vi "Create Channel.vi"(3 "no of points":u8, 5 "WheelID (if need)":u8, 7 "PlayerID":u8=1, 8 "error in (no error)":errorcluster, 9 "Channel":T2, 10 "RDB Signalname":string, 11 "Item Ref in":T1 format="%.0x") -> (0 "error out":errorcluster)   [LabVIEW 2023, in "Vires VTD System Explorer.lvlib"]
uses:
  Vires VTD System Explorer.lvlib
  <vilib>/NI VeriStand/Custom Device API/Custom Device Channel.ctl
  <vilib>/NI VeriStand/Custom Device API/Custom Device Channel Type.ctl
  <vilib>/NI VeriStand/Custom Device API/Custom Device Item Ref.ctl
  <vilib>/xnet/xnet.llb/XNET String To IO Name (Signal).vi
  Shared/Constants.vi
  <vilib>/NI VeriStand/Custom Device API/Custom Device API.lvlib
  Shared/Vires VTD Shared.lvlib
  <resource>/objmgr/xnet.rc
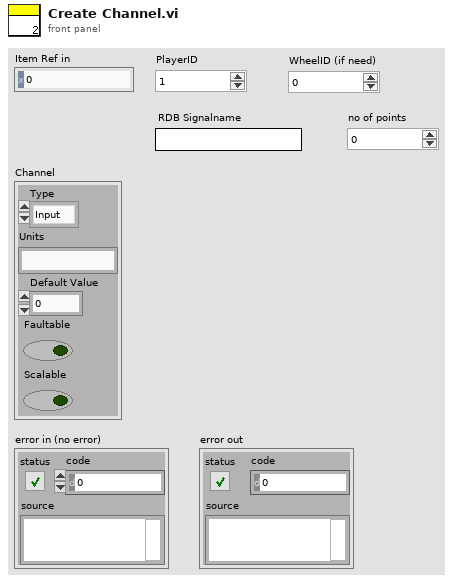
[diagram p1: front panel]
types:
  T1 = typedef "Custom Device API.lvlib/Custom Device Item Ref.ctl" = u64
  T2 = typedef "Custom Device API.lvlib/Custom Device Channel.ctl" = cluster{"Type":T3, "Units":string, "Default Value":dbl, "Faultable":bool, "Scalable":bool}
  T3 = typedef "Custom Device API.lvlib/Custom Device Channel Type.ctl" = enum16{"Input", "Output"}
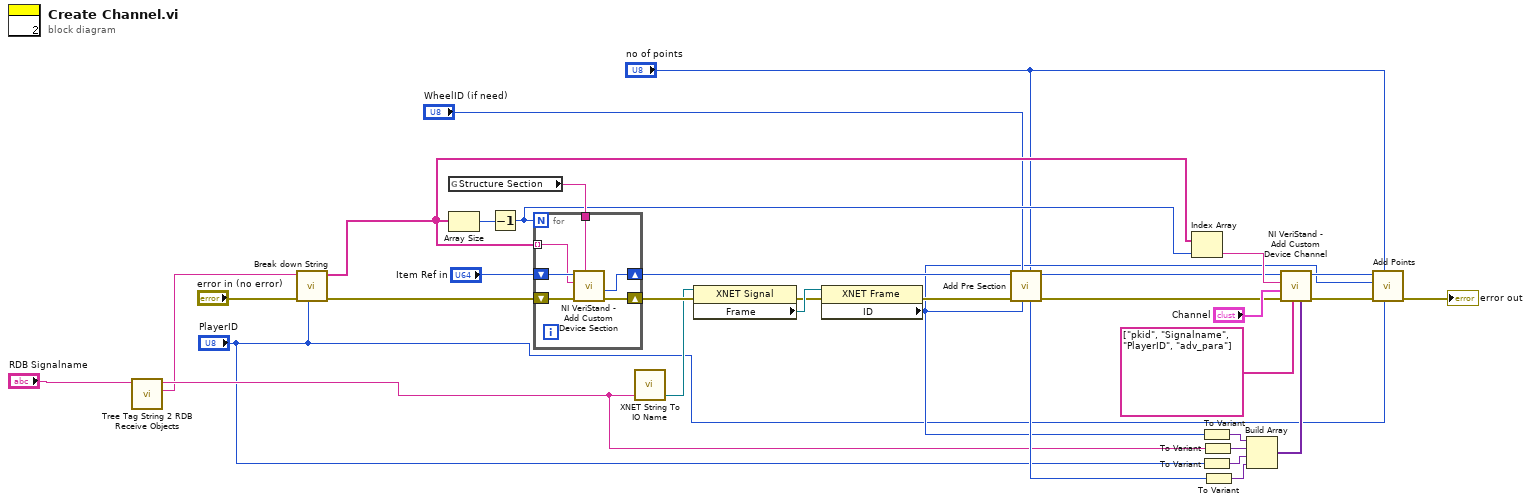
[diagram p0: block diagram]
diagram:
  n1 = call "Tree Tag String 2 RDB Receive Objects.vi"("tag string"="RDB Signalname") -> ("RDB Receive Objects"=w8:string, "RDB Signalname"=w9:string)  [unwired: 9 in]
  n2 = call "Break down String.vi"("PlayerID"="PlayerID", "Error in"="error in (no error)", "Input String"=w8) -> ("Error Out"=w30:errorcluster, "Output"=w28:string[])  [unwired: 7 in]
  n3 = global read "Constants.vi" "Structure Section"() -> (w32:string)
  n4 = Array Size(array=w28) -> (size(s)=w29:i32)
  n5 = Decrement(x=w29) -> (x-1=w27:i32)
  n6 = for {
    N: w27 -> [_]
    tunnel: w32 -> [w39]
    shift-right: [w35] -> w14
    shift-left: "Item Ref in" -> [w40]
    shift-right: [w37] -> w19
    shift-left: w30 -> [w38]
    tunnel: w28 -> [w36] mode=indexing
    n7 = call <vilib>:"NI VeriStand - Add Custom Device Section.vi"("GUID (Default Section)"=w39, "error in (no error)"=w38, "Section Name"=w36, "Parent Ref in"=w40) -> ("error out"=w37:errorcluster, "Section Ptr"=w35:T1)  [unwired: 4 in, 2 out]
  }
  n8 = call-poly <vilib>:"XNET String To IO Name.vi"("string"=w9) -> ("XNET Signal"=w18:refnum<k21>)  [unwired: 4 out]
  n9 = property class="XNET Signal"(reference=w18, error in=w19) -> (error out=w20:errorcluster, "Frame"=w21:refnum<k21>)  [unwired: 1 out]
  n10 = property class="XNET Frame"(reference=w21, error in=w20) -> (error out=w16:errorcluster, "ID"=w3:u32)  [unwired: 1 out]
  n11 = call "Add Pre Section.vi"("no of points"="no of points", "Identifier"=w3, "WheelIDorContactPointID"="WheelID (if need)", "error in (no error)"=w16, "Item Ref in"=w14) -> ("error out"=w15:errorcluster, "Item Ref out"=w13:T1, "adv para"=w11:i32)  [unwired: 4 in]
  n12 = Index Array(array=w28, index=w27) -> (element=w26:string)
  n13 = To Variant(anything=w3) -> (Variant=w17:variant)
  n14 = To Variant(anything="PlayerID") -> (Variant=w22:variant)
  n15 = To Variant(anything=w9) -> (Variant=w24:variant)
  n16 = To Variant(anything=w11) -> (Variant=w12:variant)
  n17 = Build Array(w17, w24, w22, w12) -> (w23:variant[])
  n18 = call <vilib>:"NI VeriStand - Add Custom Device Channel.vi"("Property Values"=w23, "Property names"=string[] ["pkid", "Signalname", "PlayerID", "adv_para"], "error in (no error)"=w15, "Channel"="Channel", "Channel Name"=w26, "Parent Ref in"=w13) -> ("error out"=w6:errorcluster, "Parent Ref out"=w4:T1)  [unwired: 2 in, 2 out]
  n19 = call "Add Points.vi"("PlayerID"="PlayerID", "no of points"="no of points", "error in (no error)"=w6, "Identifier"=w3, "Item Ref in"=w4) -> ("error out"=→"error out":errorcluster)  [unwired: 5 in, 1 out]
